vi "ASD BSC Graph VI.vi"(11 "Region C":cluster{"BL":dbl[], "STD":dbl[], "Count":dbl[]}) -> (0 "Count Graph":cluster{i32[], "Count":dbl[]}[](graph), 2 "STDW Graph":cluster{i32[], "Count":dbl[]}[](graph), 3 "BLW Graph":cluster{i32[], "Count":dbl[]}[](graph))   [LabVIEW 2018]
panel:
  out "Count":dbl[](array[numeric])
  out "STD":dbl[](array[numeric])
  out "BL":dbl[](array[numeric])
  out "BL Graph":cluster{i32[], dbl[]}(graph)
  out "STD Graph":cluster{i32[], dbl[]}(graph)
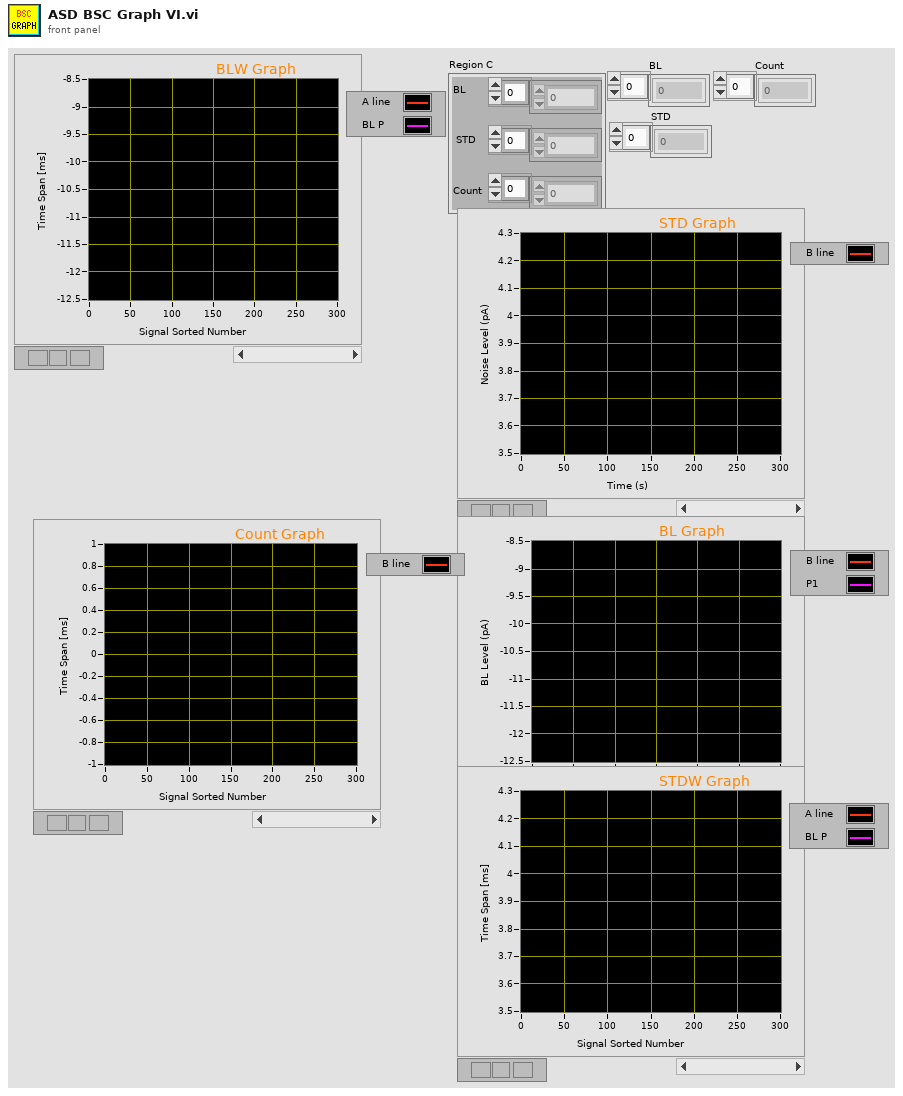
[diagram p1: front panel]
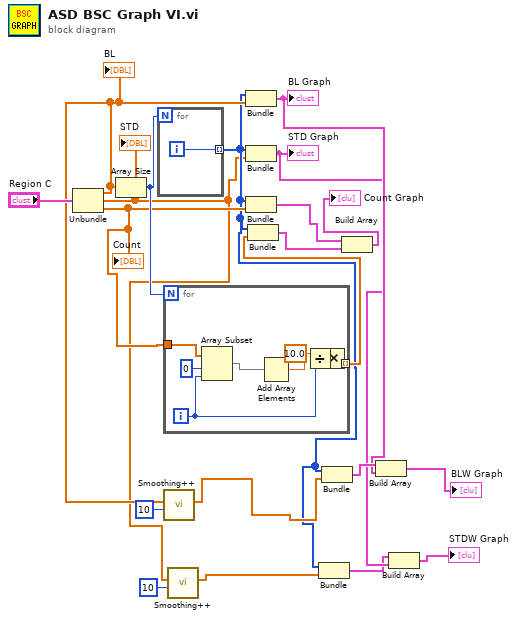
[diagram p0: block diagram]
diagram:
  n1 = Unbundle("Region C") -> ("BL"=w10:dbl[], "STD"=w3:dbl[], "Count"=w15:dbl[])
  "BL" <- w10
  "STD" <- w3
  "Count" <- w15
  n2 = Array Size(array=w10) -> (size(s)=w19:i32)
  n3 = for {
    N: w19 -> [_]
    tunnel: [w21] -> w6 mode=indexing
    i -> [w21]
  }
  n4 = for {
    N: w19 -> [_]
    tunnel: w15 -> [w29]
    tunnel: [w23] -> w17 mode=indexing
    i -> [w24]
    n5 = Array Subset(array=w29, index=0 ("指標"), length=w24) -> (w27:dbl[])
    n6 = Add Array Elements(numeric array=w27) -> (sum=w25:dbl)
    n7 = Divide(x=w25, y=w24) -> (x/y=w26:dbl)
    n8 = Multiply(x=10.0, y=w26) -> (x*y=w23:dbl)
  }
  n9 = call "Smoothing++.vi"("+/- Point"=10, "Y in"=w10) -> ("Y out"=w11:dbl[])  [unwired: 9 in]
  n10 = call "Smoothing++.vi"("+/- Point"=10, "Y in"=w3) -> ("Y out"=w2:dbl[])  [unwired: 9 in]
  n11 = Bundle(w6, "BL"=w10) -> (w8:cluster{i32[], "BL":dbl[]})  [unwired: 1 in]
  "BL Graph" <- w8
  n12 = Bundle(w6, "STD"=w3) -> (w7:cluster{i32[], "STD":dbl[]})  [unwired: 1 in]
  "STD Graph" <- w7
  n13 = Bundle(w6, "Count"=w15) -> (w13:cluster{i32[], "Count":dbl[]})  [unwired: 1 in]
  n14 = Bundle(w6, w17) -> (w16:cluster{i32[], dbl[]})  [unwired: 1 in]
  n15 = Bundle(w6, "Y out"=w2) -> (w5:cluster{i32[], "Y out":dbl[]})  [unwired: 1 in]
  n16 = Bundle(w6, "Y out"=w11) -> (w9:cluster{i32[], "Y out":dbl[]})  [unwired: 1 in]
  n17 = Build Array(w13, w16) -> (→"Count Graph":cluster{i32[], "Count":dbl[]}[])
  n18 = Build Array(w9, w8) -> (→"BLW Graph":cluster{i32[], "BL":dbl[]}[])
  n19 = Build Array(w5, w7) -> (→"STDW Graph":cluster{i32[], "STD":dbl[]}[])
